vi "Count.vi"(2 "A":dbl=1.0 format="%#_13g", 3 "S":dbl format="%#_13g") -> (0 "sqrt(x)":dbl, 1 "V":dbl)   [LabVIEW 2019]
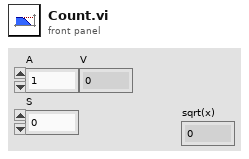
[diagram p1: front panel]
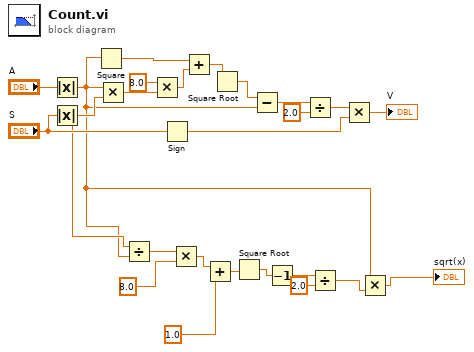
[diagram p0: block diagram]
diagram:
  n1 = Absolute Value(x="A") -> (abs(x)=w2:dbl)
  n2 = Absolute Value(x="S") -> (abs(x)=w12:dbl)
  n3 = Square(x=w2) -> (x^2=w19:dbl)
  n4 = Multiply(x=w2, y=w12) -> (x*y=w18:dbl)
  n5 = Divide(x=w12, y=w2) -> (x/y=w11:dbl)
  n6 = Multiply(x=8.0, y=w18) -> (x*y=w16:dbl)
  n7 = Sign(1:"S") -> (0:w25:dbl)
  n8 = Multiply(x=w11, y=8.0) -> (x*y=w9:dbl)
  n9 = Add(x=w19, y=w16) -> (x+y=w15:dbl)
  n10 = Add(x=w9, y=1.0) -> (x+y=w7:dbl)
  n11 = Square Root(x=w15) -> (sqrt(x)=w14:dbl)
  n12 = Square Root(x=w7) -> (sqrt(x)=w6:dbl)
  n13 = Subtract(x=w14, y=w2) -> (x-y=w22:dbl)
  n14 = Decrement(x=w6) -> (x-1=w5:dbl)
  n15 = Divide(x=w22, y=2.0) -> (x/y=w23:dbl)
  n16 = Divide(x=w5, y=2.0) -> (x/y=w3:dbl)
  n17 = Multiply(x=w23, y=w25) -> (x*y=→"V":dbl)
  n18 = Multiply(x=w2, y=w3) -> (x*y=→"sqrt(x)":dbl)
